vi "Message from Segments.vi"(8 "error in (no error)":errorcluster, 9 "Segments in":T1[](array[typedef]), 10 "Messages in":map{string, T3}(c390), 11 "ProtoParser in":refnum<class "ProtoParser.lvclass">) -> (0 "error out":errorcluster, 1 "Remaining":T1[](array[typedef]), 2 "Messages":map{string, T3}(c390), 3 "ProtoParser out":refnum<class "ProtoParser.lvclass">)   [LabVIEW 2020, in "LV-Protoc.lvlib" / "ProtoParser.lvclass"]
uses:
  ProtoParser.lvclass
  LV-Proto/Message.ctl
  LV-Proto/LV-Proto.lvlib
  LV-Proto/Field.ctl
  LV-Proto/Proto Type.ctl
  LV-Proto/Type.ctl
  Segment Type.ctl
  LV-Protoc.lvlib
  Raw Segment.ctl
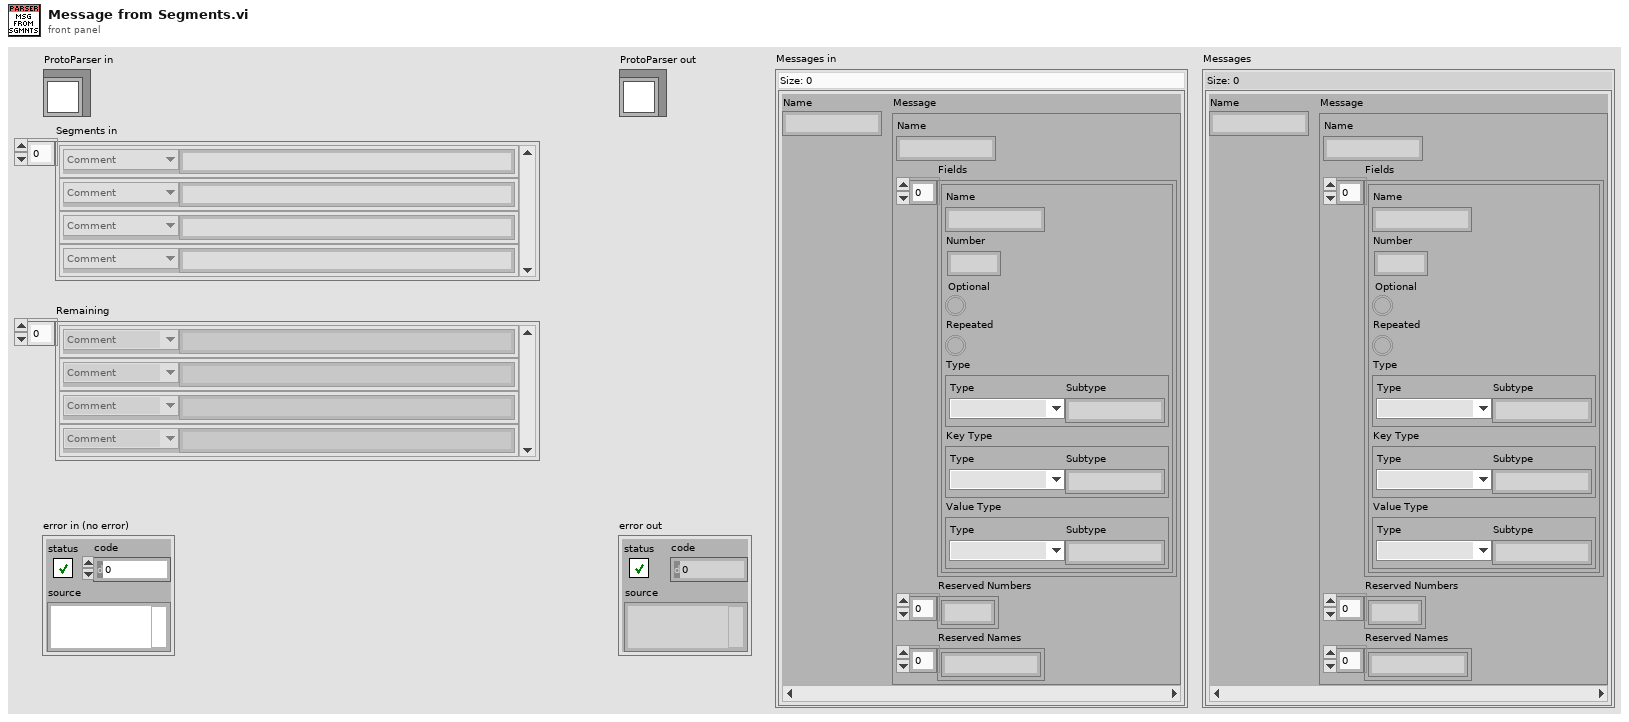
[diagram p1: front panel]
types:
  T1 = typedef "LV-Protoc.lvlib/Raw Segment.ctl" = cluster{"Type":T2, "Text":string}
  T2 = typedef "LV-Protoc.lvlib/Segment Type.ctl" = enum16{"Comment", "Message Open", "Enum Open", "Message Close", "Enum Close", "Field", "Syntax", "Import", "Enum Value", "Package", "Reserved"}
  T3 = typedef "LV-Proto.lvlib/Message.ctl" = cluster{"Name":string, "Fields":T4[], "Reserved Numbers":u32[], "Reserved Names":string[]}
  T4 = typedef "LV-Proto.lvlib/Field.ctl" = cluster{"Name":string, "Number":u32, "Optional":bool, "Repeated":bool, "Type":T5, "Key Type":T5, "Value Type":T5}
  T5 = typedef "LV-Proto.lvlib/Type.ctl" = cluster{"Type":T6, "Subtype":string}
  T6 = typedef "LV-Proto.lvlib/Proto Type.ctl" = enum16{"UNKNOWN", "double", "float", "int32", "int64", "uint32", "uint64", "sint32", "sint64", "fixed32", "fixed64", "sfixed32", "sfixed64", "bool", "string", "bytes", "enum", "map", "message"}
  T7 = typedef "LV-Protoc.lvlib/Reserved Type.ctl" = enum16{"Numeric", "Name"}
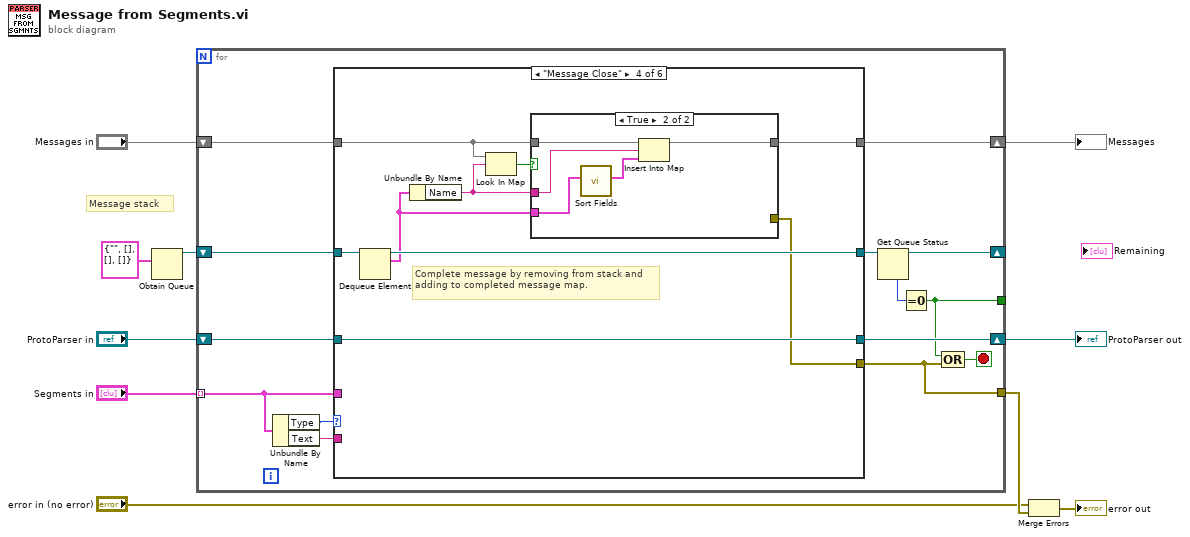
[diagram p0: block diagram]
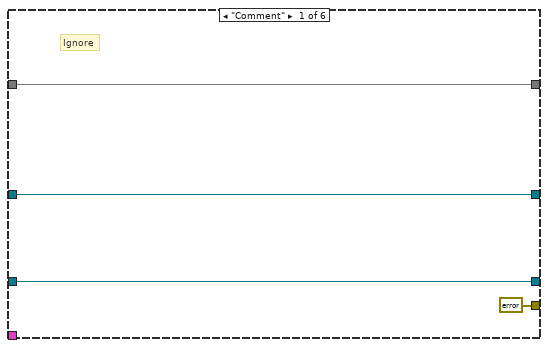
[diagram p2: hidden frame]
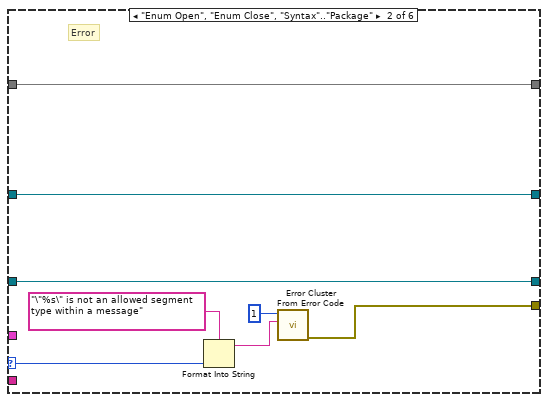
[diagram p3: hidden frame]
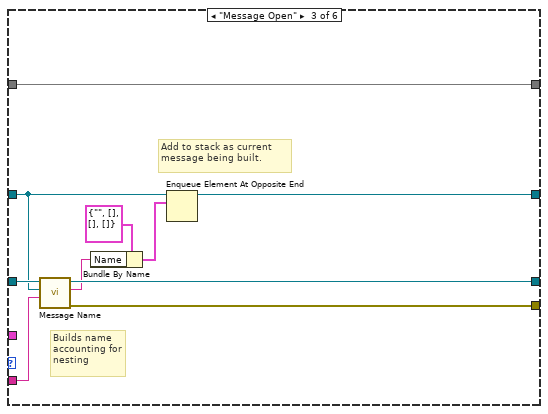
[diagram p4: hidden frame]
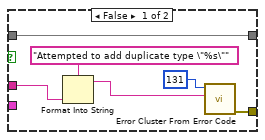
[diagram p5: hidden frame]
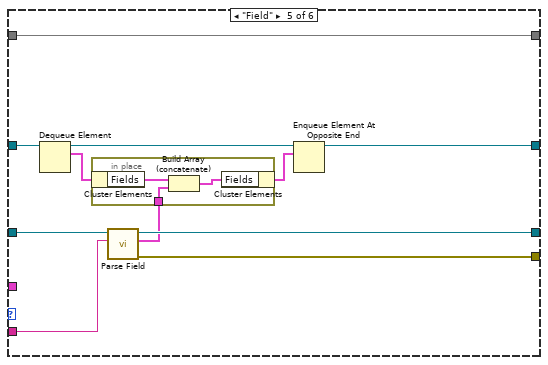
[diagram p6: hidden frame]
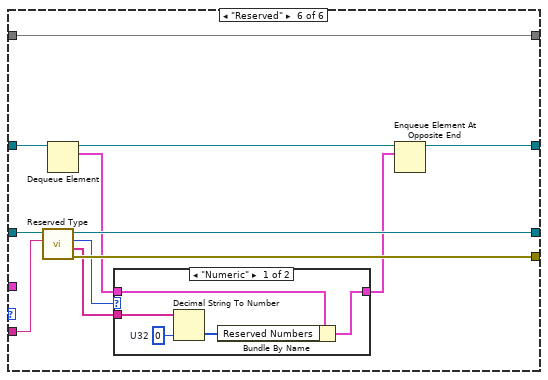
[diagram p7: hidden frame]
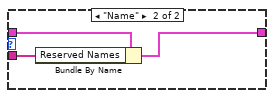
[diagram p8: hidden frame]
diagram:
  # "Message stack"
  n1 = Obtain Queue(element data type=T3 {"Name"="", "Fields"=[], "Reserved Numbers"=[], "Reserved Names"=[]} ("Message")) -> (queue out=w5:refnum<queue>)  [unwired: 4 in, 2 out]
  n2 = for {
    tunnel: "Segments in" -> [w12] mode=indexing
    shift-right: [w20] -> w10
    shift-left: "ProtoParser in" -> [w21]
    shift-right: [w15] -> _
    shift-left: w5 -> [w18]
    shift-right: [w16] -> w7
    shift-left: "Messages in" -> [w19]
    tunnel: [w13] -> _
    tunnel: [w24] -> w3
    stop <- w11 stop-if-true
    n3 = Unbundle By Name(w12) -> ("Type"=w23:T2, "Text"=w22:string)
    n4 = case shown="\"Message Close\"" w23 {
      selector: w23 -> [_ w31 _ _ _ _]
      tunnel: w22 -> [_ _ w42 _ w73 w88]
      tunnel: w12 -> [_ _ _ _ _ _]
      tunnel: w21 -> [w28 w36 w46 w55 w77 w91]
      tunnel: [w28 w36 w44 w55 w74 w89] -> w20
      tunnel: w19 -> [w26 w34 w45 w51 w75 w90]
      tunnel: w18 -> [w27 w35 w43 w54 w76 w85]
      tunnel: [w27 w35 w39 w53 w69 w82] -> w17
      tunnel: [w26 w34 w45 w48 w75 w90] -> w16
      tunnel: [errorcluster {"status"=FALSE, "code"=0, "source"=""} ("error out") w33 w37 w47 w67 w92] -> w24
      frame "Comment" {
        # "Ignore"
      }
      frame "Enum Open", "Enum Close", "Syntax".."Package" {
        # "Error"
        n5 = Format Into String(format string="\"%s\" is not an allowed segment type within a message", w31) -> (resulting string=w30:string)  [unwired: 2 in, 1 out]
        n6 = call <vilib>:"Error Cluster From Error Code.vi"("error message (\"\")"=w30, "error code (0)"=1) -> ("error out"=w33:errorcluster)  [unwired: 7 in]
      }
      frame "Message Open" {
        # "Add to stack as current message being built."
        # "Builds name accounting for nesting"
        n7 = call "Message Name.vi"("Text"=w42, "Message Stack in"=w43, "ProtoParser in"=w46) -> ("error out"=w37:errorcluster, "Message Name"=w40:string, "ProtoParser out"=w44:refnum<class "ProtoParser.lvclass">)  [unwired: 6 in]
        n8 = Bundle By Name(cluster=T3 {"Name"="", "Fields"=[], "Reserved Numbers"=[], "Reserved Names"=[]} ("Message"), "Name"=w40) -> (w38:T3)
        n9 = Enqueue Element At Opposite End(queue=w43, element=w38) -> (queue out=w39:refnum<queue>)  [unwired: 2 in, 2 out]
      }
      frame "Message Close" {
        # "Complete message by removing from stack and adding to completed message map."
        n10 = Dequeue Element(queue=w54) -> (queue out=w53:refnum<queue>, element=w49:T3)  [unwired: 2 in, 2 out]
        n11 = Unbundle By Name(w49) -> ("Name"=w50:string)
        n12 = Look In Map(map=w51, key=w50) -> (key not found?=w52:bool)  [unwired: 1 in, 1 out]
        n13 = case shown="True" w52 {
          tunnel: w51 -> [w61 w66]
          tunnel: w50 -> [w59 w65]
          tunnel: w49 -> [_ w64]
          tunnel: [w61 w63] -> w48
          tunnel: [w56 _] -> w47
          frame False {
            n14 = Format Into String(format string="Attempted to add duplicate type \"%s\"", w59) -> (resulting string=w57:string)  [unwired: 2 in, 1 out]
            n15 = call <vilib>:"Error Cluster From Error Code.vi"("error message (\"\")"=w57, "error code (0)"=131) -> ("error out"=w56:errorcluster)  [unwired: 7 in]
          }
          frame True {
            n16 = call "Sort Fields.vi"("Message in"=w64) -> ("Message"=w62:T3)  [unwired: 10 in]
            n17 = Insert Into Map(map in=w66, key=w65, value=w62) -> (map out=w63:map{string, T3})  [unwired: 2 out]
          }
        }
      }
      frame "Field" {
        n18 = Dequeue Element(queue=w76) -> (queue out=w72:refnum<queue>, element=w71:T3)  [unwired: 2 in, 2 out]
        n19 = call "Parse Field.vi"("Text"=w73, "ProtoParser in"=w77) -> ("error out"=w67:errorcluster, "Field"=w70:T4, "ProtoParser out"=w74:refnum<class "ProtoParser.lvclass">)  [unwired: 7 in]
        n20 = in-place {
          in-place-border: w70 -> [w79]
          n21 = in-place-cluster #1(w71) -> ("Fields"=w80:T4[])
          n22 = Build Array (concatenate)(w80, w79) -> (w78:T4[])
          n23 = in-place-cluster #1("Fields"=w78) -> (w68:T3)
        }
        n24 = Enqueue Element At Opposite End(queue=w72, element=w68) -> (queue out=w69:refnum<queue>)  [unwired: 2 in, 2 out]
      }
      frame "Reserved" {
        n25 = call "Reserved Type.vi"("Text"=w88, "ProtoParser in"=w91) -> ("error out"=w92:errorcluster, "Values"=w86:string[], "Reserved Type"=w87:T7, "ProtoParser out"=w89:refnum<class "ProtoParser.lvclass">)  [unwired: 6 in]
        n26 = Dequeue Element(queue=w85) -> (queue out=w83:refnum<queue>, element=w84:T3)  [unwired: 2 in, 2 out]
        n27 = case shown="\"Numeric\"" w87 {
          tunnel: w86 -> [w97 w99]
          tunnel: w84 -> [w93 w100]
          tunnel: [w94 w98] -> w81
          frame "Numeric" {
            w95 = u32 0  # U32
            n28 = Decimal String To Number(string=w97, default (0L)=w95) -> (number=w96:u32[])  [unwired: 1 in, 1 out]
            n29 = Bundle By Name(cluster=w93, "Reserved Numbers"=w96) -> (w94:T3)
          }
          frame "Name" {
            n30 = Bundle By Name(cluster=w100, "Reserved Names"=w99) -> (w98:T3)
          }
        }
        n31 = Enqueue Element At Opposite End(queue=w83, element=w81) -> (queue out=w82:refnum<queue>)  [unwired: 2 in, 2 out]
      }
    }
    n32 = Get Queue Status(queue=w17) -> (queue out=w15:refnum<queue>, # elements in queue=w14:i32)  [unwired: 2 in, 6 out]
    n33 = Equal To 0?(x=w14) -> (x = 0?=w13:bool)
    n34 = Compound Arithmetic op=OR(w13, w24) -> (w11:bool)
  }
  "ProtoParser out" <- w10
  "Messages" <- w7
  n35 = Merge Errors("error in (no error)", w3) -> (→"error out":errorcluster)
